vi "fsm_pluto_sequence_test.vi"() -> ()   [LabVIEW 2026]
uses:
  types/TestConfig.ctl
  <vilib>/Analysis/4window.llb/Hanning Window (DBL).vi
  <vilib>/Analysis/baseanly.llb/Mean (DBL).vi
  <vilib>/Analysis/2dsp.llb/Complex FFT.vi
  <vilib>/Analysis/4window.llb/AllCosWindow (DBL).vi
  <vilib>/Python/Open Venv Python Session.vi
  <vilib>/Analysis/1siggen.llb/Ramp Pattern by Samples.vi
  <vilib>/Analysis/NI_AALBase.lvlib
  <vilib>/Analysis/NI_AALPro.lvlib
panel:
  out "Received Signal \n Hann Windowed Spectrum":cluster{"Ramp Pattern":dbl[], dbl[]}(graph)
  out "Hann FFT Magnitude \nSpectrum (Normalized)":dbl[](array[numeric])
  out "Hann FFT Magnitude \nSpectrum (Centered)":dbl[](array[numeric])
  out "Hann FFT Magnitude\nSpectrum (Raw)":dbl[](array[numeric])
  out "Hann FFT \nComplex Spectrum":cdb[](array[numeric])
  out "Hann Windowed \nComplex Samples":cdb[](array[numeric])
  out "Windowed Q Samples":dbl[](array[numeric])
  out "Windowed I Samples":dbl[](array[numeric])
  out "FFT Magnitude Spectrum (Normalized)":dbl[](array[numeric])
  out "Received Signal \n Frequency Spectrum":cluster{"Ramp Pattern":dbl[], dbl[]}(graph)
  out "Frequency Axis (Mhz)":dbl[](array[numeric])
  out "FFT Magnitude Spectrum (Centered).":dbl[](array[numeric])
  out "N":i32
  out "FFT Magnitude Spectrum (Raw).":dbl[](array[numeric])
  out "FFT Complex Spectrum":cdb[](array[numeric])
  out "Raw Complex Samples":cdb[](array[numeric])
  out "Crest Factor (dB) indicator":dbl
  out "Crest Factor Valid":bool
  out "Crest Factor":dbl
  out "Peak Complex Magnitude":dbl
  out "Q RMS.":dbl
  out "I RMS.":dbl
  out "Q mean - DC offset":dbl format="%0.2f"
  out "I mean - DC offset":dbl format="%0.2f"
  out "Raw Q Samples":dbl[](array[numeric])
  out "Raw I Samples":dbl[](array[numeric])
  out "Sequence Index":i32
  out "Test Finished":bool
  out "Sequence Available":bool
  out "size(s)":i32
  out "Selected Configuration":T1
  in  "Test Sequence":T2(array[cluster])
  out "error out":errorcluster
  out "Acquisition Valid":bool
  out "Processing Valid":bool
  out "RMS Is Finite?":bool
  in  "Requested Samples":u32
  out "Capture Status":string
  out "Capture Configuration":string
  out "Error Status":string
  out "Resolved Log Path":path
  in  "Log File":path
  out "Log Record":string
  out "Log Status":string
  out "Processed Result":dbl
  out "Captured Data":dbl[](array[numeric])
  in  "Start Test":bool
  out "Current State":T3(ring)
  out "Configuration Status":string
  in  "Gain (dB)":dbl
  in  "Sample Rate (Ms/s)":dbl
  in  "Test Freq (Mhz)":dbl
  in  "stop":bool
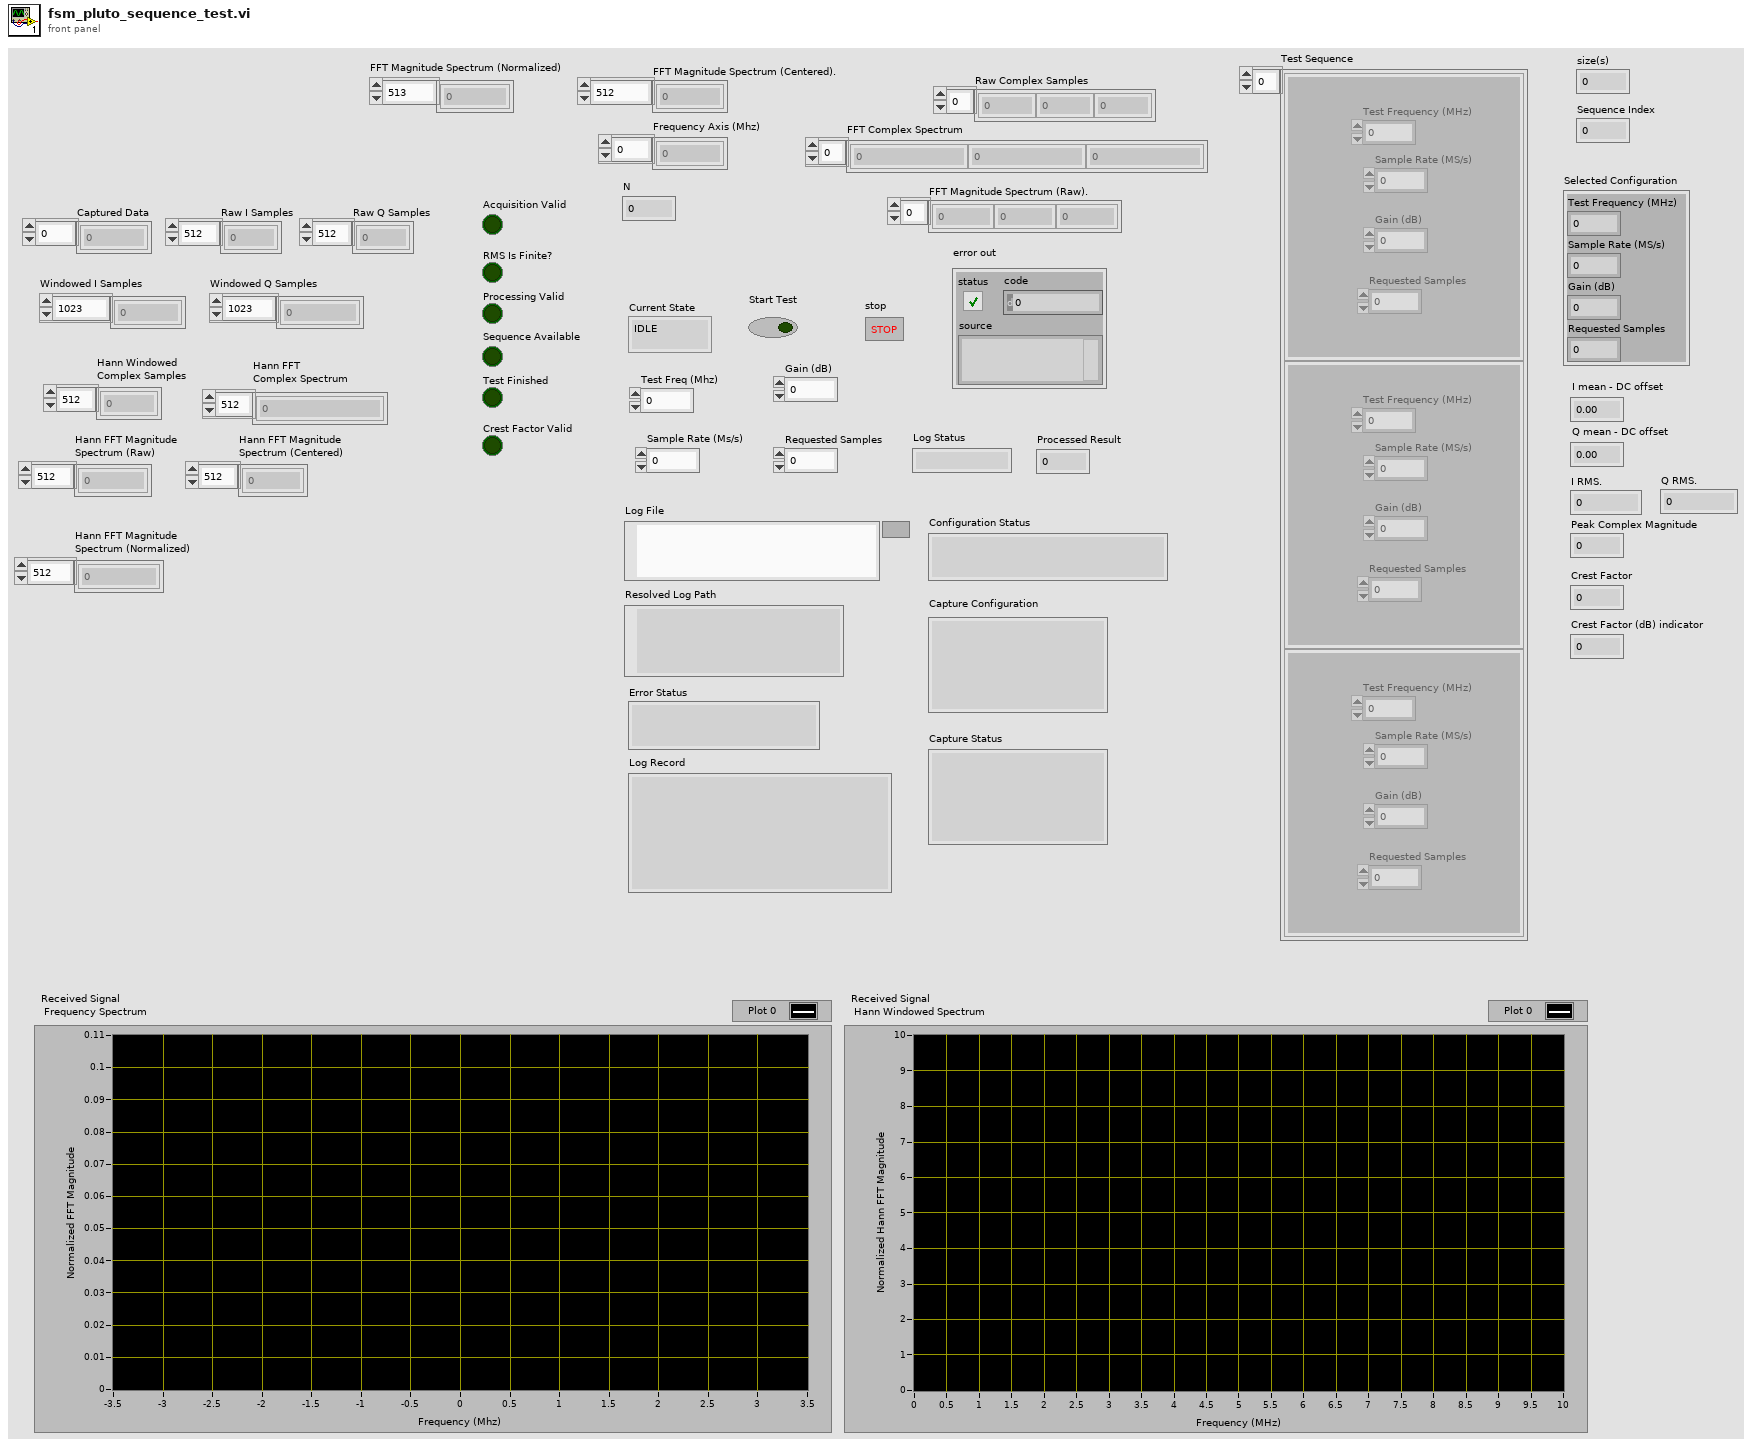
[diagram p1: front panel]
types:
  T1 = cluster{"Test Frequency (MHz)":dbl, "Sample Rate (MS/s)":dbl, "Gain (dB)":dbl, "Requested Samples":u32}
  T2 = cluster{"Test Frequency (MHz)":dbl, "Sample Rate (MS/s)":dbl, "Gain (dB)":dbl, "Requested Samples":u32}[]
  T3 = enum16{"IDLE", "CONFIGURE", "CAPTURE", "PROCESS", "LOG ", "ERROR "}
  T4 = cluster{"Acquisition Status":string, "Processing Status":string, "Overall Status":string, "Received Samples":u32, "RMS Value":dbl, "RMS Valid":bool, "Error Details":string}
  T5 = typedef "TestConfig.ctl" = cluster{"Test Frequency (Mhz)":dbl, "Sample Rate (Ms/s)":dbl, "Gain (dB)":dbl, "Requested Samples":u32}
  T6 = enum16{"open", "replace", "create", "open or create", "replace or create", "replace or create with confirmation"}
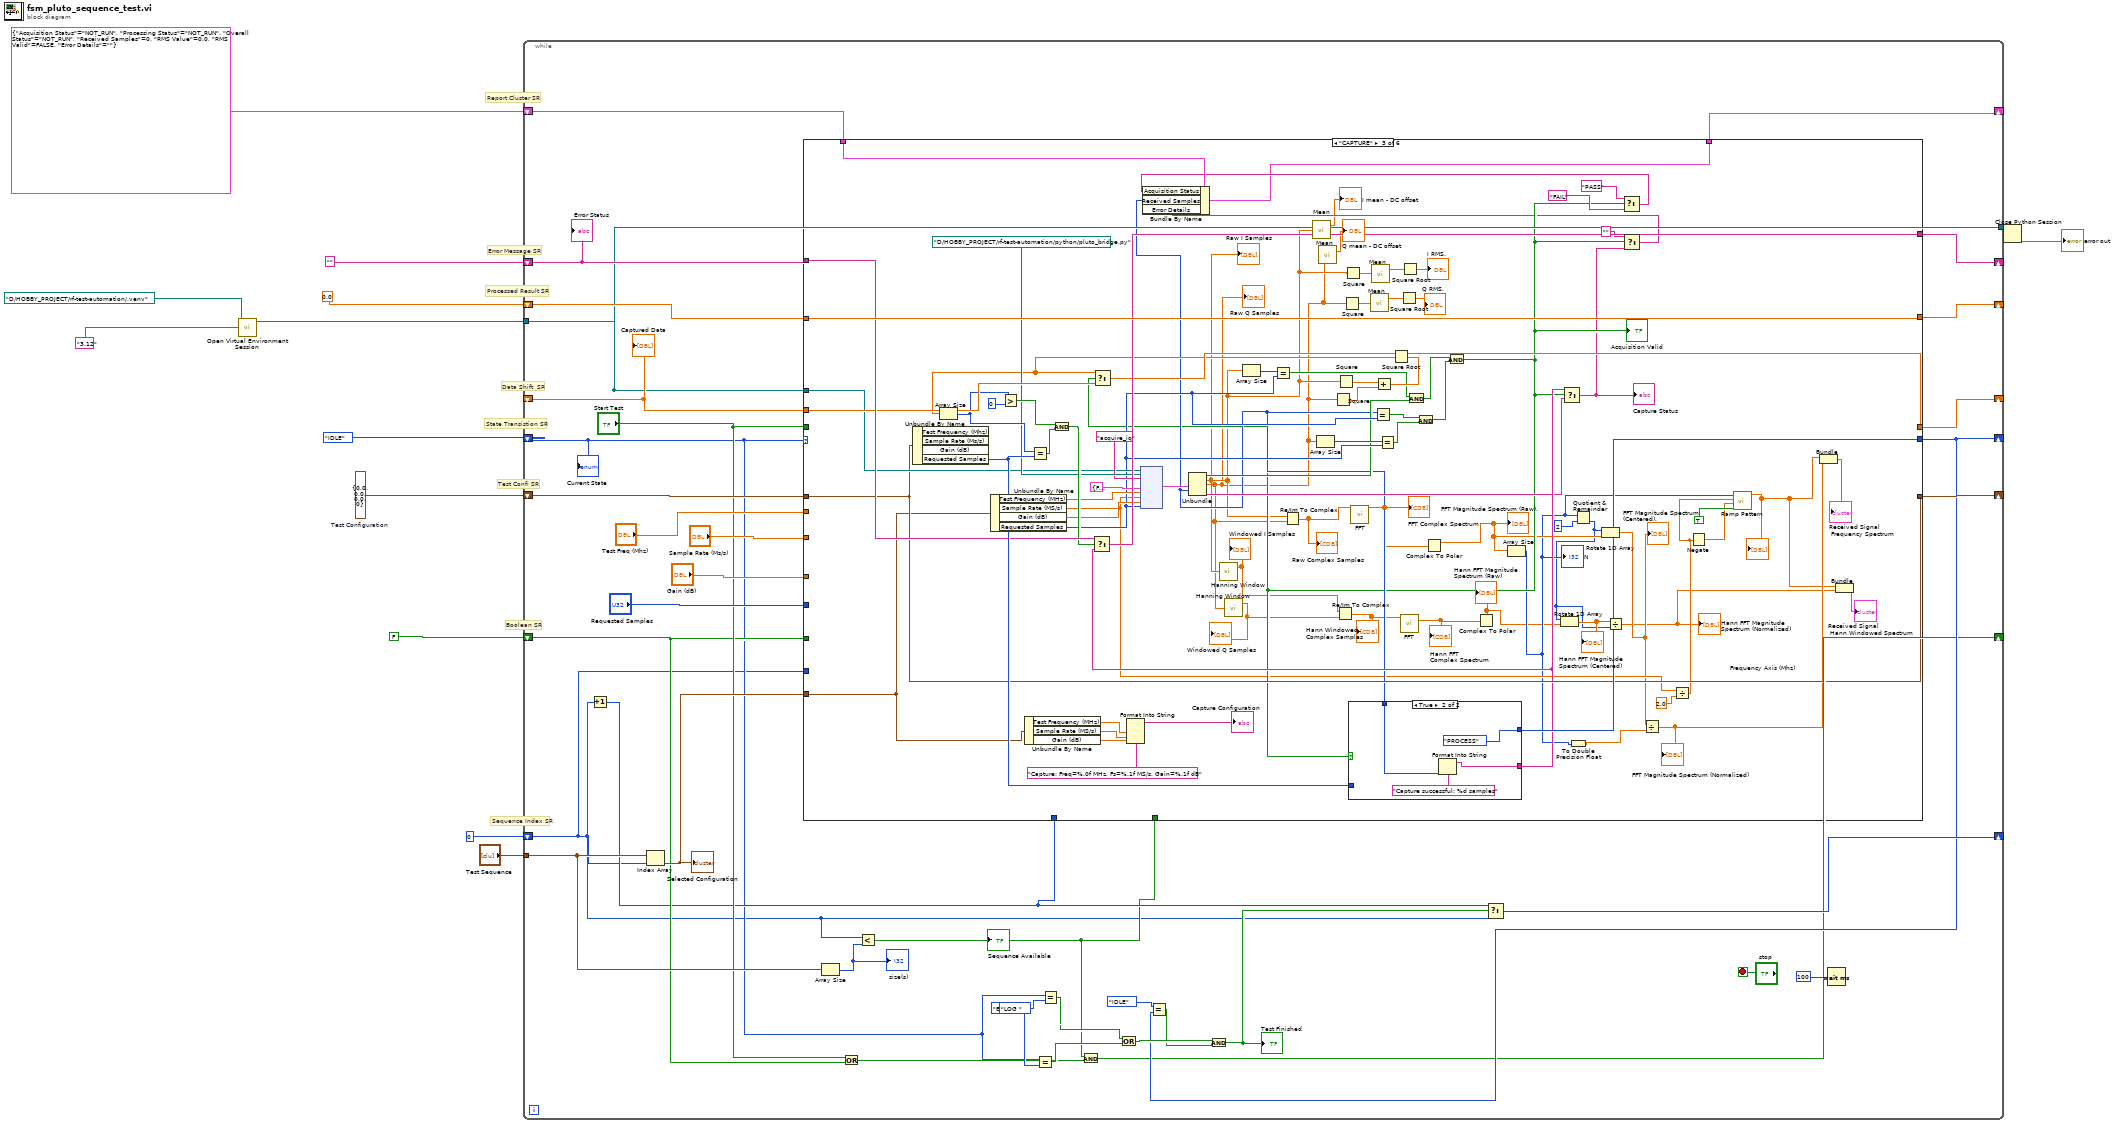
[diagram p0: block diagram]
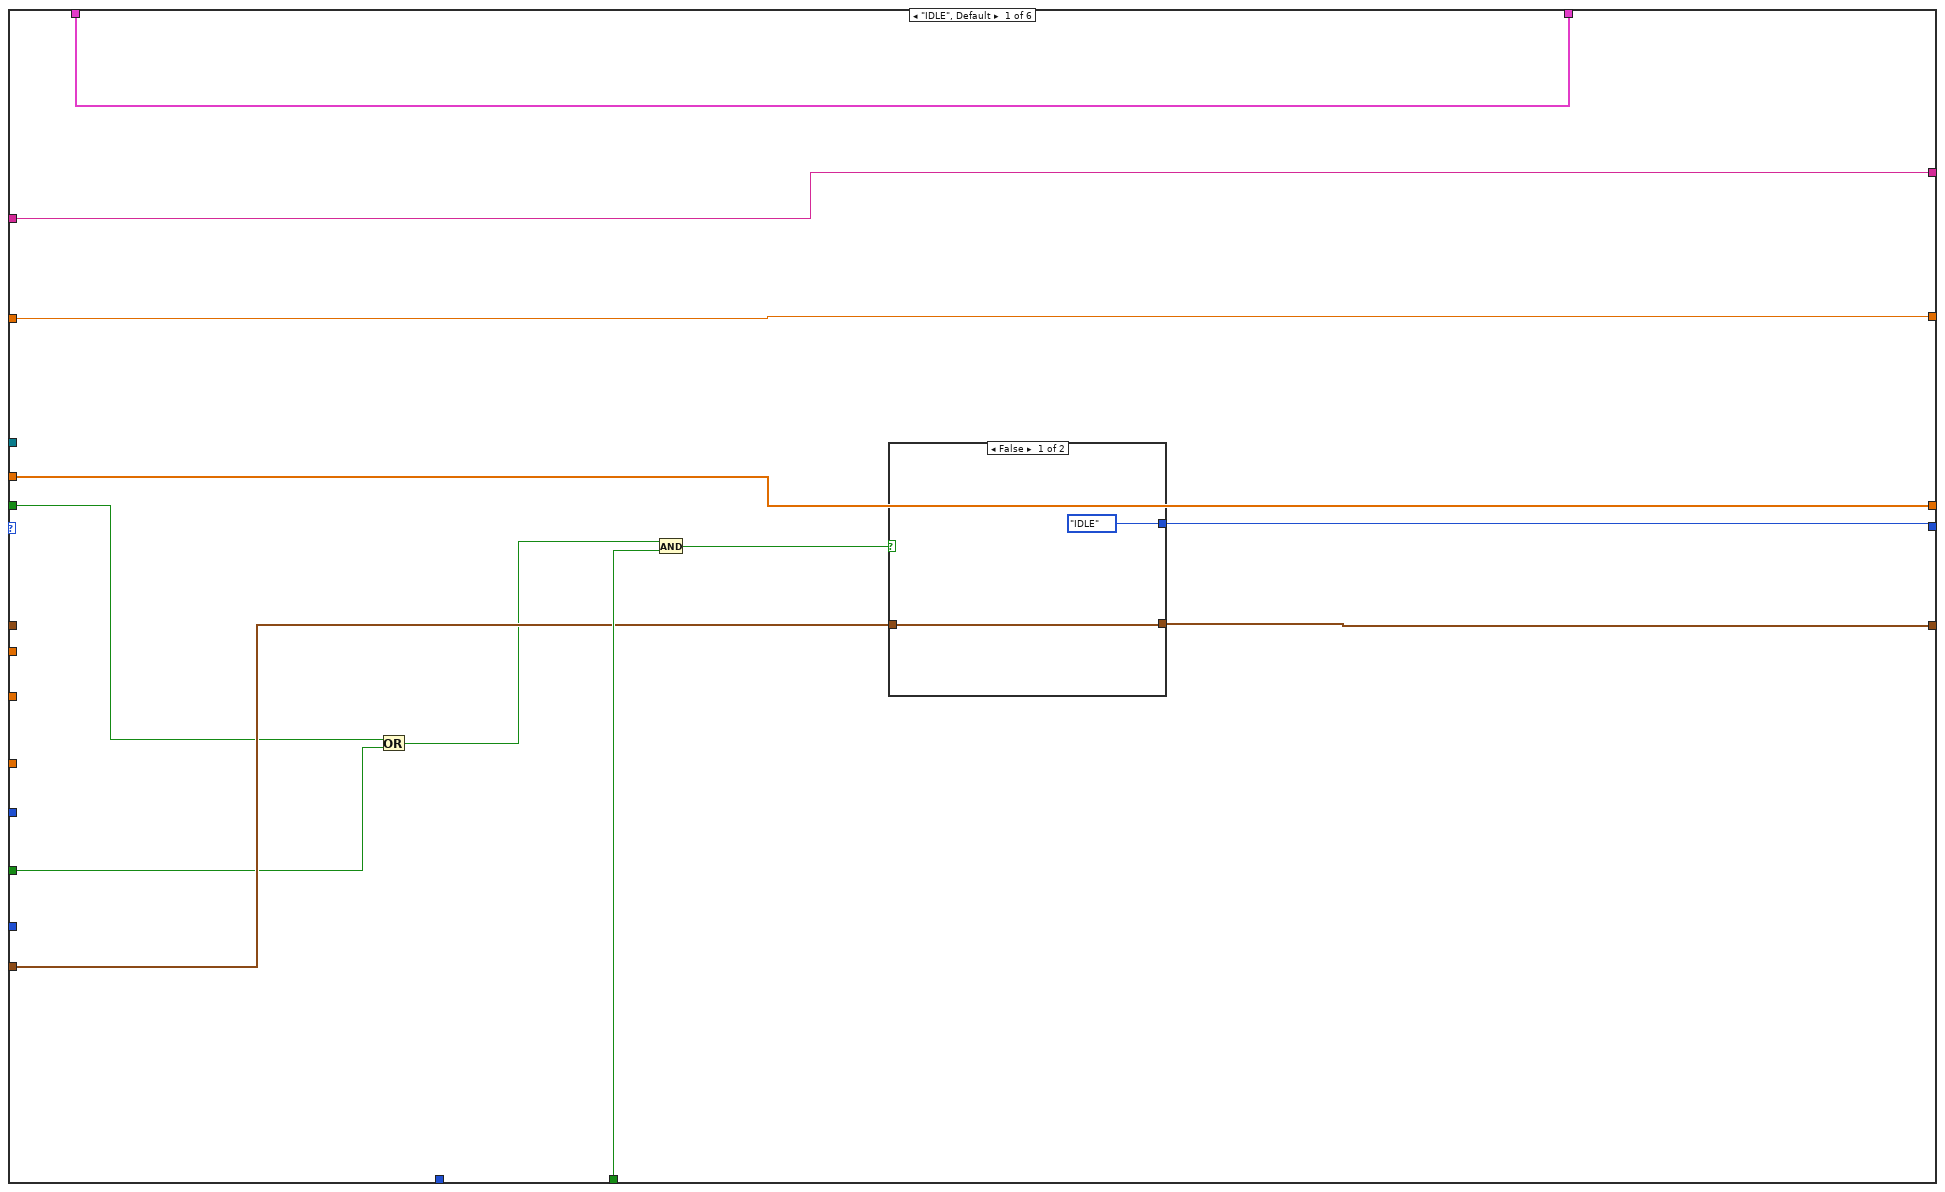
[diagram p2: hidden frame]
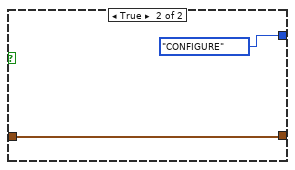
[diagram p3: hidden frame]
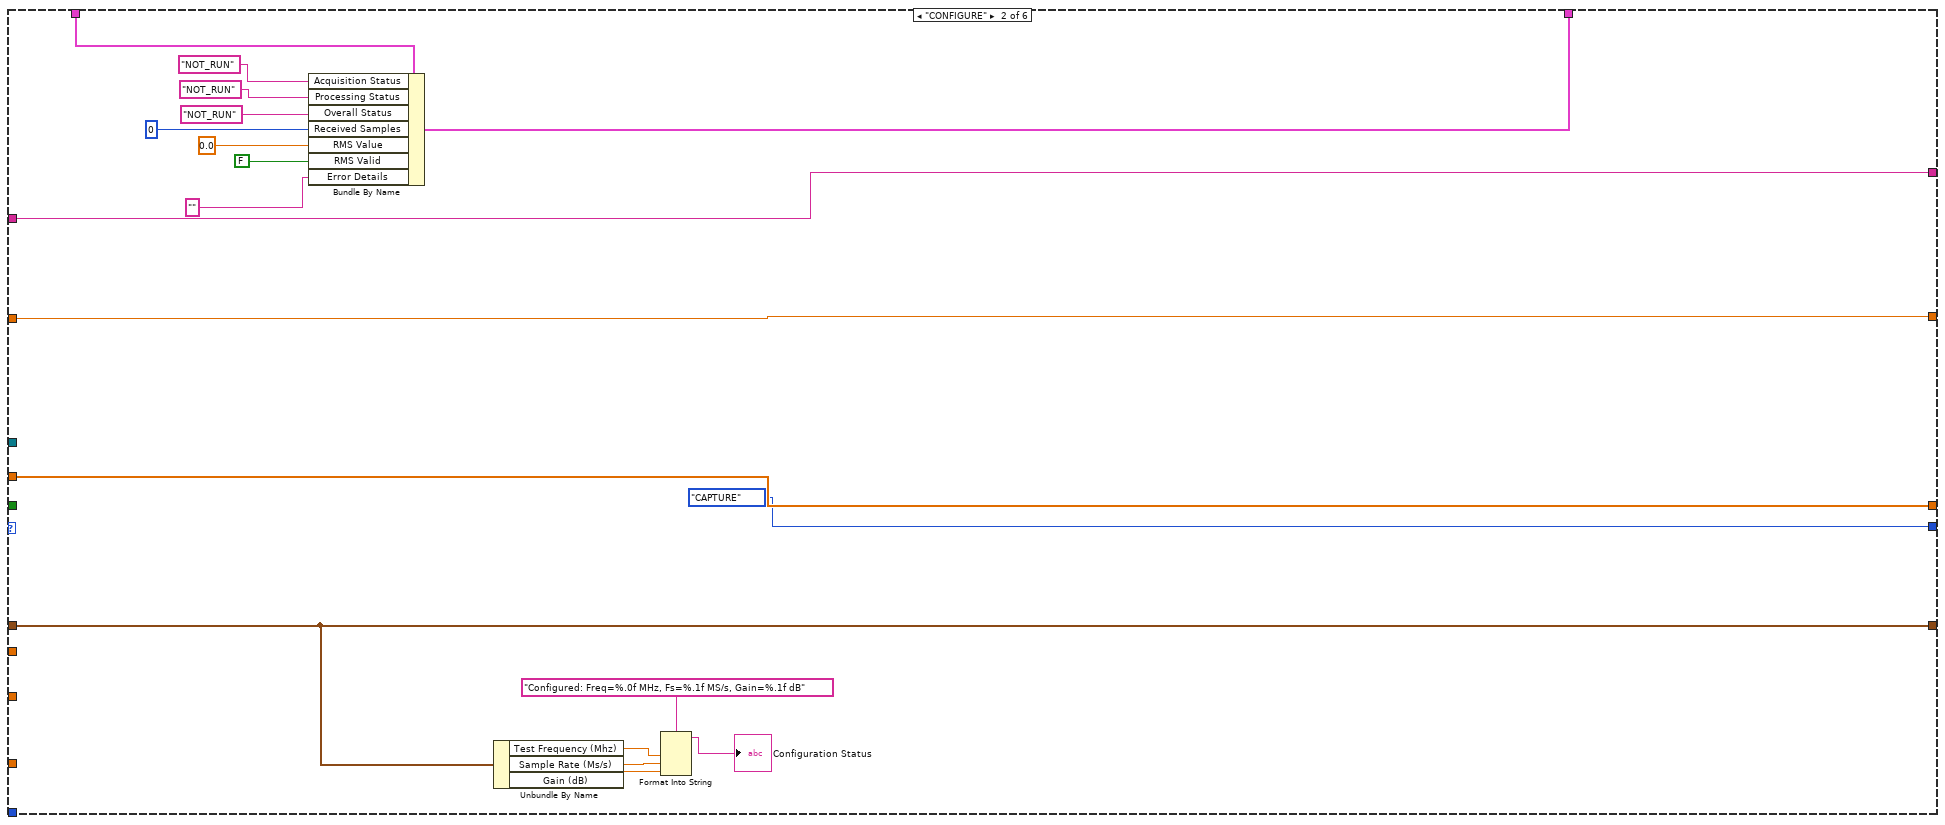
[diagram p4: hidden frame]
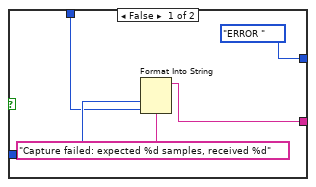
[diagram p5: hidden frame]
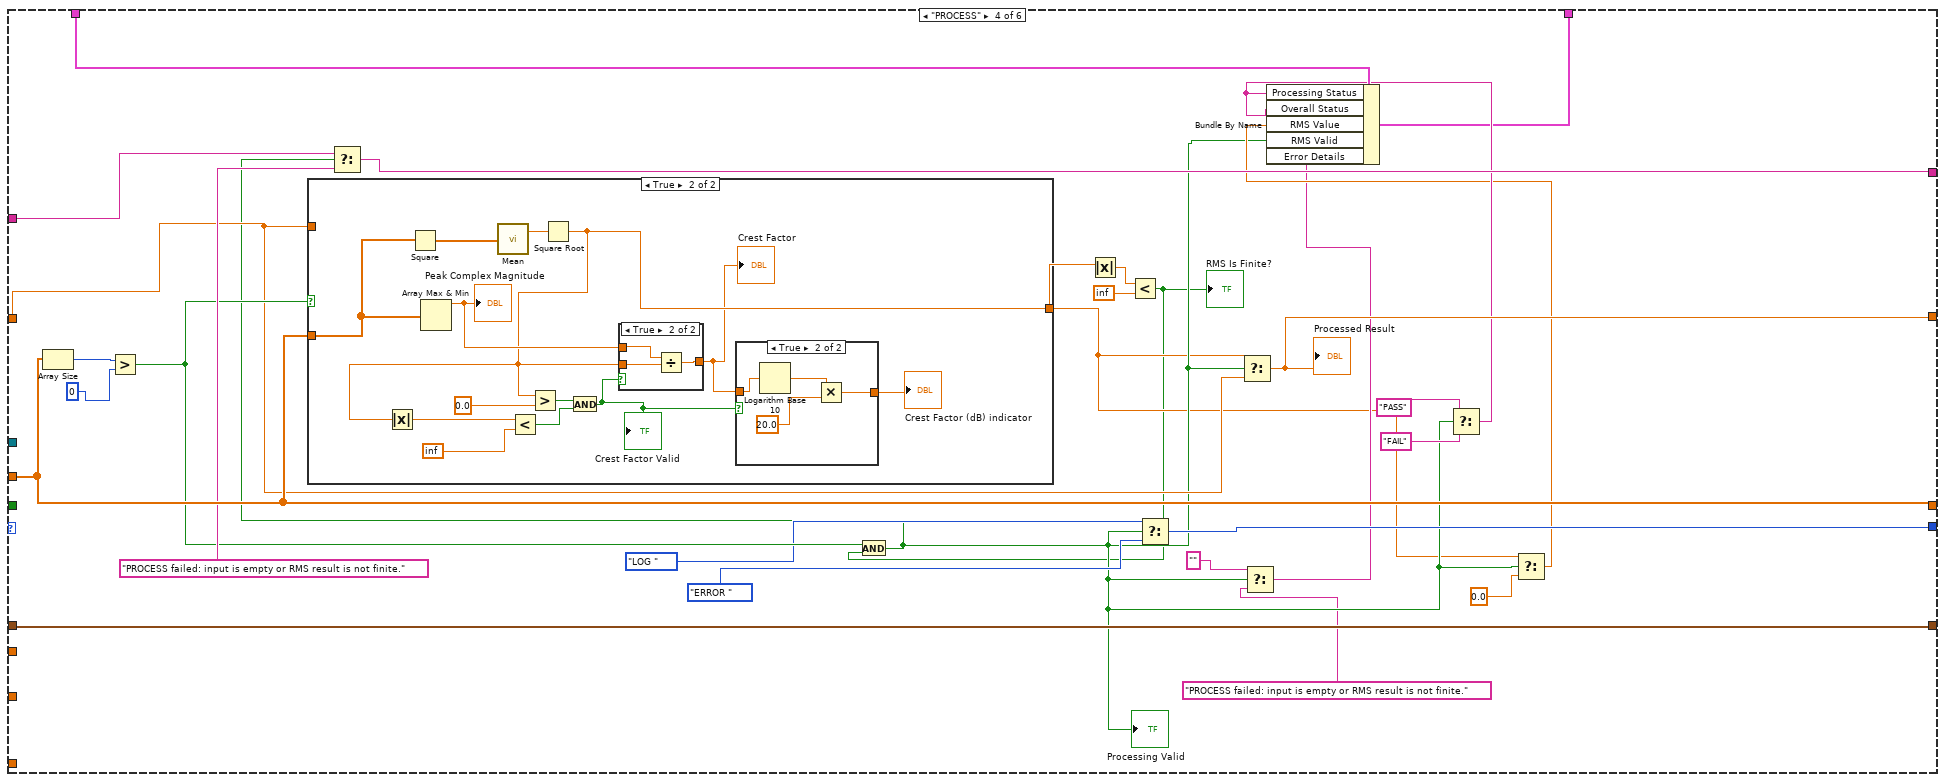
[diagram p6: hidden frame]
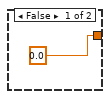
[diagram p8: hidden frame]
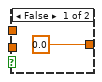
[diagram p9: hidden frame]
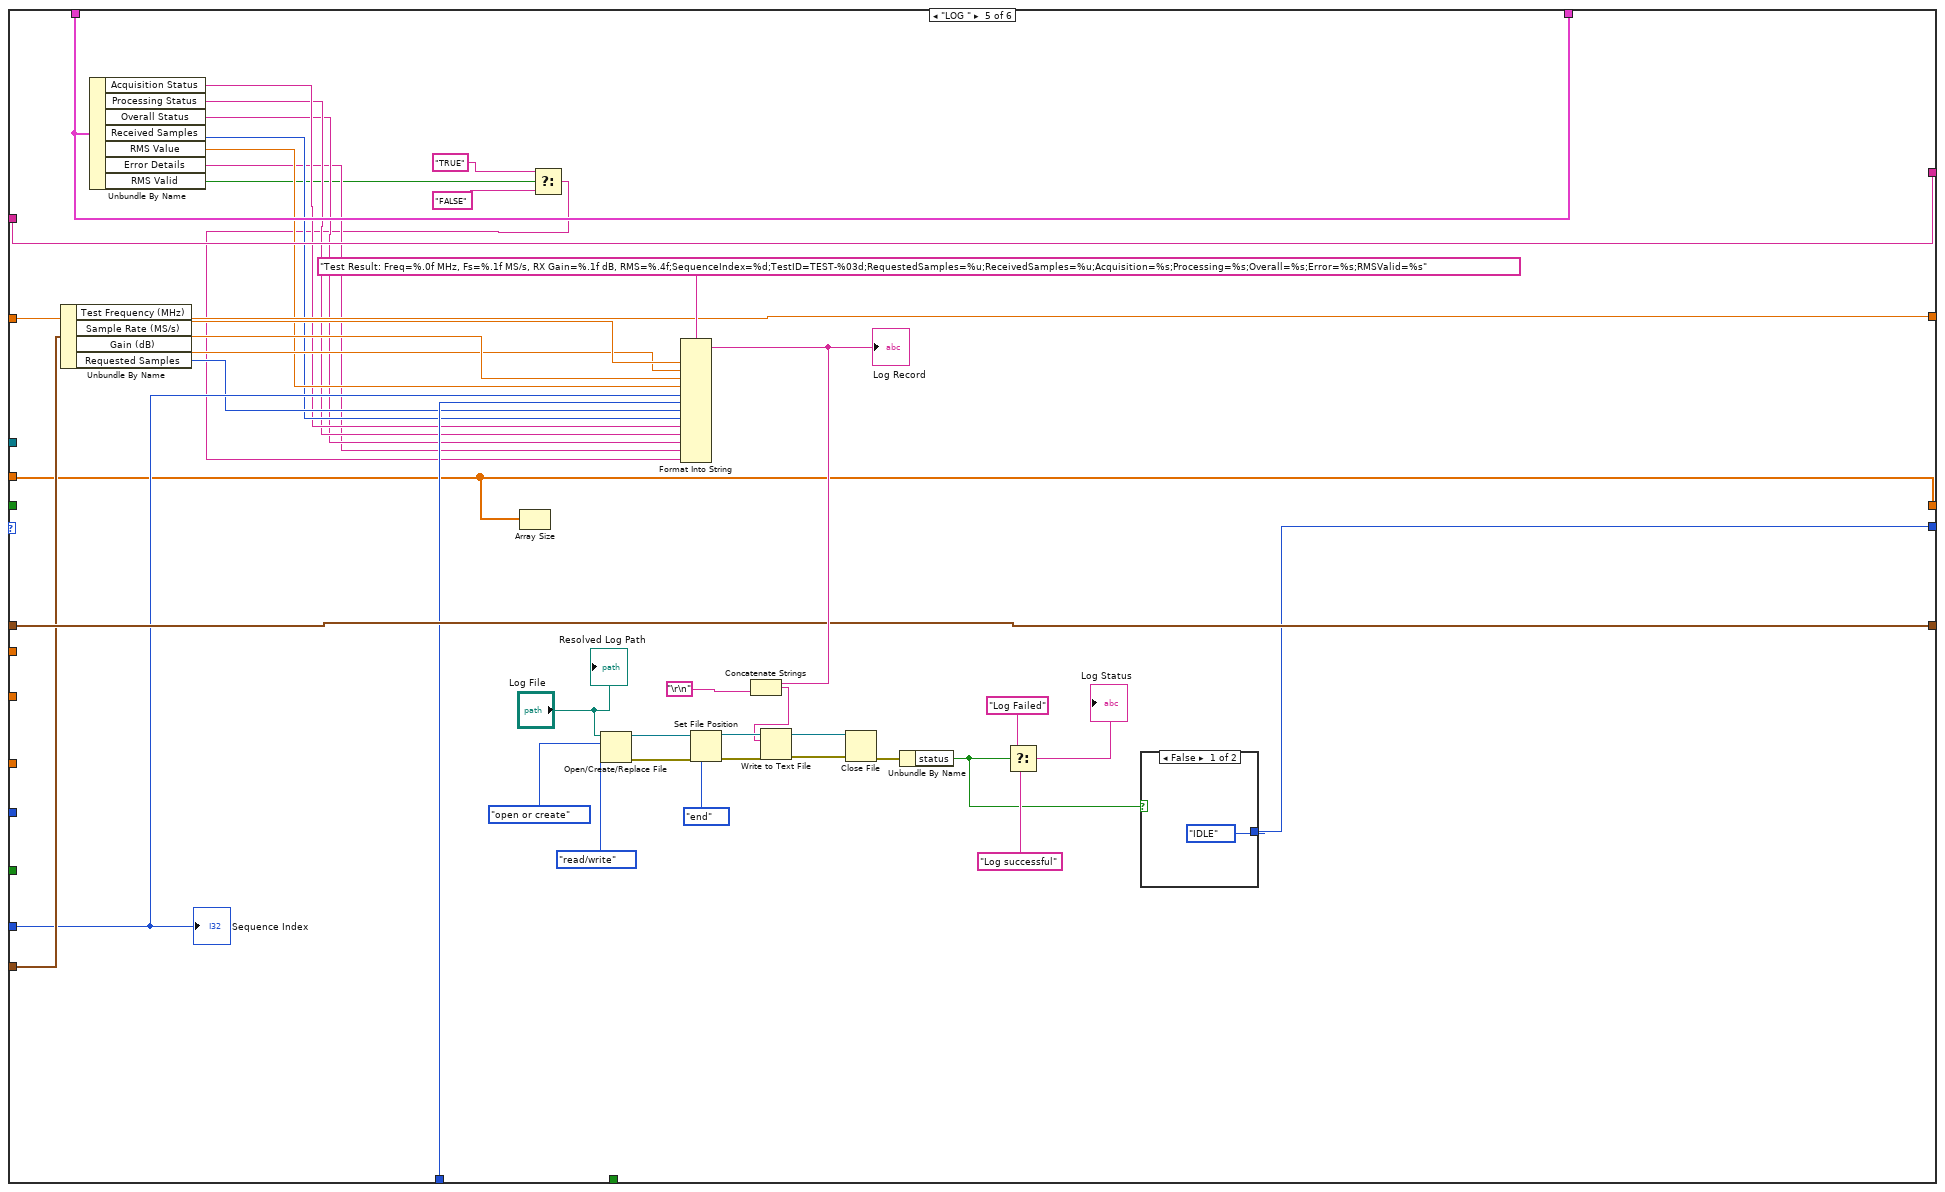
[diagram p10: hidden frame]
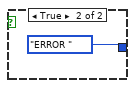
[diagram p11: hidden frame]
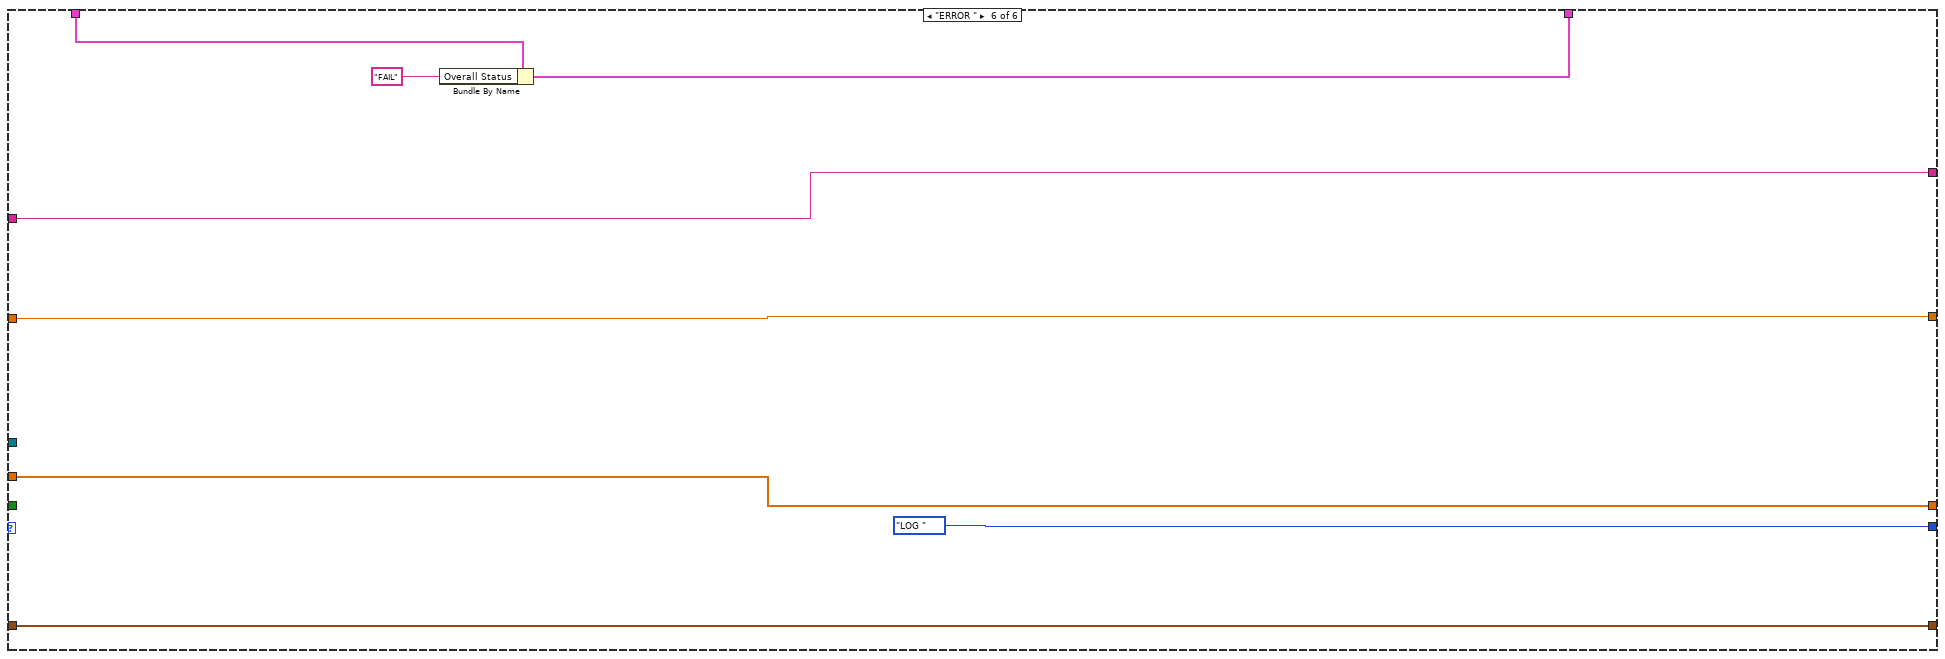
[diagram p12: hidden frame]
diagram:
  w10 = T5 {"Test Frequency (Mhz)"=0.0, "Sample Rate (Ms/s)"=0.0, "Gain (dB)"=0.0, "Requested Samples"=0}  # Test Configuration
  # "Sequence Index SR"
  # "Boolean SR"
  # "Test Confi SR"
  # "State Transistion SR"
  # "Data Shift  SR"
  # "Processed Result SR"
  # "Error Message SR"
  # "Report Cluster SR"
  n1 = call-poly <vilib>:"Open Virtual Environment Session.vi"("Python version"="3.12", "Env path"=path "D:/HOBBY_PROJECT/rf-test-automation/.venv") -> ("session out"=w7:refnum<k35>)  [unwired: 8 in, 1 out]
  n2 = while {
    shift-right: [w25] -> _
    shift-left: T3."IDLE" -> [w16]
    shift-right: [w49] -> _
    shift-left: _ -> [w48]
    shift-right: [w47] -> _
    shift-left: 0.0 -> [w46]
    shift-right: [w42] -> _
    shift-left: "" -> [w41]
    shift-right: [w39] -> _
    shift-left: w10 -> [w40]
    tunnel: w7 -> [w37]
    tunnel: [w37] -> w6
    shift-right: [w35] -> _
    shift-left: u32 0 -> [w14]
    tunnel: "Test Sequence" -> [w34]
    shift-right: [w21] -> _
    shift-left: FALSE -> [w23]
    shift-right: [w19] -> _
    shift-left: T4 {"Acquisition Status"="NOT_RUN", "Processing Status"="NOT_RUN", "Overall Status"="NOT_RUN", "Received Samples"=0, "RMS Value"=0.0, "RMS Valid"=FALSE, "Error Details"=""} -> [w18]
    stop <- "stop" stop-if-true
    n3 = Increment(x=w14) -> (x+1=w20:u32)
    n4 = Index Array(array=w34, index=w14) -> (element=w36:T1)
    "Selected Configuration" <- w36
    n5 = Array Size(array=w34) -> (size(s)=w33:i32)
    "size(s)" <- w33
    n6 = Or(x="Start Test", y=w23) -> (x .or. y?=w22:bool)
    n7 = Less?(x=w14, y=w33) -> (x < y?=w15:bool)
    "Sequence Available" <- w15
    n8 = case shown="\"CAPTURE\"" w16 {
      tunnel: "Test Freq (Mhz)" -> [_ _ _ _ _ _]
      tunnel: "Sample Rate (Ms/s)" -> [_ _ _ _ _ _]
      tunnel: "Gain (dB)" -> [_ _ _ _ _ _]
      tunnel: "Start Test" -> [w54 _ _ _ _ _]
      tunnel: [w63 w84 w160 w207 w243 w283] -> w49
      tunnel: w48 -> [w63 w84 w161 w207 w243 w283]
      tunnel: [w62 w83 w171 w196 w272 w282] -> w47
      tunnel: w46 -> [w62 w83 w171 w195 w272 w282]
      tunnel: [w61 T3."CAPTURE" w165 w197 w247 T3."LOG "] -> w25
      tunnel: [w60 w81 w162 w202 w253 w279] -> w42
      tunnel: w41 -> [w60 w81 w163 w204 w253 w279]
      tunnel: w40 -> [_ w80 w150 w208 w252 w280]
      tunnel: [w59 w80 w150 w208 w252 w280] -> w39
      tunnel: "Requested Samples" -> [_ _ _ _ _ _]
      tunnel: w37 -> [_ _ w151 _ _ _]
      tunnel: w36 -> [w56 _ w131 _ w251 _]
      tunnel: w15 -> [w57 _ _ _ _ _]
      tunnel: w23 -> [w55 _ _ _ _ _]
      tunnel: w14 -> [_ _ _ _ w246 _]
      tunnel: w20 -> [_ _ _ _ w245 _]
      tunnel: w18 -> [w52 w76 w130 w193 w242 w278]
      tunnel: [w52 w75 w121 w183 w242 w277] -> w19
      frame "IDLE", Default {
        n9 = Or(x=w54, y=w55) -> (x .or. y?=w53:bool)
        n10 = And(x=w53, y=w57) -> (x .and. y?=w58:bool)
        n11 = case shown="False" w58 {
          tunnel: [T3."IDLE" T3."CONFIGURE"] -> w61
          tunnel: [w64 w66] -> w59
          tunnel: w56 -> [w64 w66]
          frame False {
          }
          frame True {
          }
        }
      }
      frame "CONFIGURE" {
        n12 = Bundle By Name(cluster=w76, "Acquisition Status"="NOT_RUN", "Processing Status"="NOT_RUN", "Overall Status"="NOT_RUN", "Received Samples"=0, "RMS Value"=0.0, "RMS Valid"=FALSE, "Error Details"="") -> (w75:T4)
        n13 = Unbundle By Name(w80) -> ("Test Frequency (Mhz)"=w79:dbl, "Sample Rate (Ms/s)"=w78:dbl, "Gain (dB)"=w77:dbl)
        n14 = Format Into String(format string="Configured: Freq=%.0f MHz, Fs=%.1f MS/s, Gain=%.1f dB", w79, w78, w77) -> (resulting string=→"Configuration Status":string)  [unwired: 2 in, 1 out]
      }
      frame "CAPTURE" {
        n15 = Unbundle By Name(w150) -> ("Requested Samples"=w164:u32)  [unwired: 3 out]
        n16 = Unbundle By Name(w131) -> ("Test Frequency (MHz)"=w149:dbl, "Sample Rate (MS/s)"=w108:dbl, "Gain (dB)"=w148:dbl, "Requested Samples"=w141:u32)
        n17 = Unbundle By Name(w131) -> ("Test Frequency (MHz)"=w169:dbl, "Sample Rate (MS/s)"=w168:dbl, "Gain (dB)"=w167:dbl)
        n18 = Format Into String(format string="Capture: Freq=%.0f MHz, Fs=%.1f MS/s, Gain=%.1f dB", w169, w168, w167) -> (resulting string=→"Capture Configuration":string)  [unwired: 2 in, 1 out]
        n19 = node(w151, path "D:/HOBBY_PROJECT/rf-test-automation/python/pluto_bridge.py" ("module path"), "acquire_iq" ("function name"), cluster{bool, dbl[], dbl[], i32, string} {FALSE, [], [], 0, ""}, w149, w108, w148, w141) -> (w147:cluster{bool, dbl[], dbl[], i32, string})  [unwired: 5 in, 4 out]
        n20 = Unbundle(w147) -> (w139:bool, w98:dbl[], w97:dbl[], w126:i32, w132:string)
        "Raw I Samples" <- w98
        "Raw Q Samples" <- w97
        n21 = call-poly <vilib>:"Hanning Window.vi"("X"=w98) -> ("Windowed X"=w96:dbl[])  [unwired: 1 out]
        "Windowed I Samples" <- w96
        n22 = call-poly <vilib>:"Hanning Window.vi"("X"=w97) -> ("Windowed X"=w95:dbl[])  [unwired: 1 out]
        "Windowed Q Samples" <- w95
        n23 = Array Size(array=w98) -> (size(s)=w142:i32)
        n24 = Equal?(x=w142, y=w141) -> (x = y?=w140:bool)
        n25 = Re/Im To Complex(1:w97, 2:w98) -> (0:w112:cdb[])
        "Raw Complex Samples" <- w112
        n26 = call-poly <vilib>:"Mean.vi"("X"=w98) -> ("mean"=→"I mean - DC offset":dbl)  [unwired: 1 out]
        n27 = Array Size(array=w97) -> (size(s)=w143:i32)
        n28 = call-poly <vilib>:"Mean.vi"("X"=w97) -> ("mean"=→"Q mean - DC offset":dbl)  [unwired: 1 out]
        n29 = Square(x=w97) -> (x^2=w146:dbl[])
        n30 = Re/Im To Complex(1:w95, 2:w96) -> (0:w94:cdb[])
        "Hann Windowed \nComplex Samples" <- w94
        n31 = Square(x=w98) -> (x^2=w145:dbl[])
        n32 = Square(x=w97) -> (x^2=w117:dbl[])
        n33 = Square(x=w98) -> (x^2=w116:dbl[])
        n34 = call-poly <vilib>:"FFT.vi"("X"=w112) -> ("FFT {X}"=w111:cdb[])  [unwired: 9 in, 1 out]
        "FFT Complex Spectrum" <- w111
        n35 = call-poly <vilib>:"Mean.vi"("X"=w117) -> ("mean"=w115:dbl)  [unwired: 1 out]
        n36 = call-poly <vilib>:"Mean.vi"("X"=w116) -> ("mean"=w118:dbl)  [unwired: 1 out]
        n37 = Equal?(x=w126, y=w141) -> (x = y?=w138:bool)
        n38 = Add(x=w145, y=w146) -> (x+y=w144:dbl[])
        n39 = Equal?(x=w143, y=w141) -> (x = y?=w137:bool)
        n40 = Square Root(x=w144) -> (sqrt(x)=w134:dbl[])
        n41 = Array Size(array=w134) -> (size(s)=w156:i32)
        n42 = Greater?(x=w156, y=0) -> (0:w159:bool)
        n43 = Equal?(x=w156, y=w164) -> (x = y?=w158:bool)
        n44 = And(x=w159, y=w158) -> (x .and. y?=w157:bool)
        n45 = Square Root(x=w115) -> (sqrt(x)=→"Q RMS.":dbl)
        n46 = call-poly <vilib>:"FFT.vi"("X"=w94) -> ("FFT {X}"=w93:cdb[])  [unwired: 9 in, 1 out]
        "Hann FFT \nComplex Spectrum" <- w93
        n47 = Square Root(x=w118) -> (sqrt(x)=→"I RMS.":dbl)
        n48 = And(x=w140, y=w139) -> (x .and. y?=w136:bool)
        n49 = And(x=w138, y=w137) -> (x .and. y?=w135:bool)
        n50 = Complex To Polar(r * e^(i*theta)=w111) -> (r=w110:dbl[])  [unwired: 1 out]
        "FFT Magnitude Spectrum (Raw)." <- w110
        n51 = And(x=w136, y=w135) -> (x .and. y?=w125:bool)
        "Acquisition Valid" <- w125
        n52 = Select(t=w134, s=w125, f=w161) -> (s? t:f=w160:dbl[])
        n53 = case shown="True" w125 {
          tunnel: [T3."ERROR " T3."PROCESS"] -> w165
          tunnel: w164 -> [w174 _]
          tunnel: [w173 w179] -> w133
          tunnel: w126 -> [w172 w177]
          frame False {
            n54 = Format Into String(format string="Capture failed: expected %d samples, received %d", w174, w172) -> (resulting string=w173:string)  [unwired: 2 in, 1 out]
          }
          frame True {
            n55 = Format Into String(format string="Capture successful: %d samples", w177) -> (resulting string=w179:string)  [unwired: 2 in, 1 out]
          }
        }
        n56 = Select(t=w163, s=w157, f=w133) -> (s? t:f=w162:string)
        n57 = Complex To Polar(r * e^(i*theta)=w93) -> (r=w92:dbl[])  [unwired: 1 out]
        "Hann FFT Magnitude\nSpectrum (Raw)" <- w92
        n58 = Array Size(array=w110) -> (size(s)=w101:i32)
        "N" <- w101
        n59 = Select(t=w133, s=w125, f=w132) -> (s? t:f=w123:string)
        "Capture Status" <- w123
        n60 = To Double Precision Float(number=w101) -> (double precision float=w100:dbl)
        n61 = Quotient & Remainder(x=w101, y=2) -> (floor(x/y)=w90:i32)  [unwired: 1 out]
        n62 = Rotate 1D Array(1:w92, 2:w90) -> (0:w91:dbl[])
        "Hann FFT Magnitude \nSpectrum (Centered)" <- w91
        n63 = Rotate 1D Array(1:w110, 2:w90) -> (0:w103:dbl[])
        "FFT Magnitude Spectrum (Centered)." <- w103
        n64 = Divide(x=w91, y=w90) -> (x/y=w88:dbl[])
        "Hann FFT Magnitude \nSpectrum (Normalized)" <- w88
        n65 = Select(t="PASS", s=w125, f="FAIL") -> (s? t:f=w127:string)
        n66 = Select(t="", s=w125, f=w123) -> (s? t:f=w122:string)
        n67 = Bundle By Name(cluster=w130, "Acquisition Status"=w127, "Received Samples"=w126, "Error Details"=w122) -> (w121:T4)
        n68 = Divide(x=w103, y=w100) -> (x/y=w99:dbl[])
        "FFT Magnitude Spectrum (Normalized)" <- w99
        n69 = Divide(x=w108, y=2.0) -> (x/y=w102:dbl)
        n70 = Negate(x=w102) -> (-x=w105:dbl)
        n71 = call-poly <vilib>:"Ramp Pattern.vi"("exclude end?"=TRUE, "start"=w105, "end"=w102, "samples"=w101) -> ("Ramp Pattern"=w89:dbl[])  [unwired: 6 in, 1 out]
        "Frequency Axis (Mhz)" <- w89
        n72 = Bundle("Ramp Pattern"=w89, w99) -> (→"Received Signal \n Frequency Spectrum":cluster{"Ramp Pattern":dbl[], dbl[]})  [unwired: 1 in]
        n73 = Bundle("Ramp Pattern"=w89, w88) -> (→"Received Signal \n Hann Windowed Spectrum":cluster{"Ramp Pattern":dbl[], dbl[]})  [unwired: 1 in]
      }
      frame "PROCESS" {
        n74 = Array Size(array=w207) -> (size(s)=w206:i32)
        n75 = Greater?(x=w206, y=0) -> (0:w200:bool)
        n76 = case shown="True" w200 {
          tunnel: [w209 w213] -> w182
          tunnel: w207 -> [_ w220]
          tunnel: w195 -> [w209 _]
          frame False {
          }
          frame True {
            n77 = Square(x=w220) -> (x^2=w222:dbl[])
            n78 = Array Max & Min(array=w220) -> (max value=w214:dbl)  [unwired: 3 out]
            "Peak Complex Magnitude" <- w214
            n79 = call-poly <vilib>:"Mean.vi"("X"=w222) -> ("mean"=w221:dbl)  [unwired: 1 out]
            n80 = Square Root(x=w221) -> (sqrt(x)=w213:dbl)
            n81 = Absolute Value(x=w213) -> (abs(x)=w217:dbl)
            n82 = Less?(x=w217, y=inf) -> (x < y?=w215:bool)
            n83 = Greater?(x=w213, y=0.0) -> (0:w218:bool)
            n84 = And(x=w218, y=w215) -> (x .and. y?=w212:bool)
            "Crest Factor Valid" <- w212
            n85 = case shown="True" w212 {
              tunnel: w214 -> [_ w231]
              tunnel: w213 -> [_ w230]
              tunnel: [0.0 w229] -> w211
              frame False {
              }
              frame True {
                n86 = Divide(x=w231, y=w230) -> (x/y=w229:dbl)
              }
            }
            "Crest Factor" <- w211
            n87 = case shown="True" w212 {
              tunnel: w211 -> [_ w227]
              tunnel: [0.0 w224] -> w210
              frame False {
              }
              frame True {
                n88 = Logarithm Base 10(1:w227) -> (0:w226:dbl)
                n89 = Multiply(x=w226, y=20.0) -> (x*y=w224:dbl)
              }
            }
            "Crest Factor (dB) indicator" <- w210
          }
        }
        n90 = Absolute Value(x=w182) -> (abs(x)=w201:dbl)
        n91 = Less?(x=w201, y=inf) -> (x < y?=w181:bool)
        "RMS Is Finite?" <- w181
        n92 = And(x=w200, y=w181) -> (x .and. y?=w187:bool)
        "Processing Valid" <- w187
        n93 = Select(t=w204, s=w187, f="PROCESS failed: input is empty or RMS result is not finite.") -> (s? t:f=w202:string)
        n94 = Select(t=T3."LOG ", s=w187, f=T3."ERROR ") -> (s? t:f=w197:T3)
        n95 = Select(t=w182, s=w187, f=w195) -> (s? t:f=w196:dbl)
        "Processed Result" <- w196
        n96 = Select(t="" ("f"), s=w187, f="PROCESS failed: input is empty or RMS result is not finite.") -> (s? t:f=w184:string)
        n97 = Select(t="PASS" ("f"), s=w187, f="FAIL") -> (s? t:f=w190:string)
        n98 = Select(t=w182, s=w187, f=0.0) -> (s? t:f=w188:dbl)
        n99 = Bundle By Name(cluster=w193, "Processing Status"=w190, "Overall Status"=w190, "RMS Value"=w188, "RMS Valid"=w187, "Error Details"=w184) -> (w183:T4)
      }
      frame "LOG " {
        n100 = Unbundle By Name(w251) -> ("Test Frequency (MHz)"=w249:dbl, "Sample Rate (MS/s)"=w248:dbl, "Gain (dB)"=w250:dbl, "Requested Samples"=w244:u32)
        n101 = Unbundle By Name(w242) -> ("Acquisition Status"=w239:string, "Processing Status"=w238:string, "Overall Status"=w237:string, "Received Samples"=w240:u32, "RMS Value"=w241:dbl, "Error Details"=w236:string, "RMS Valid"=w235:bool)
        n102 = Array Size(array=w243) -> ()  [unwired: 1 out]
        n103 = Select(t="TRUE", s=w235, f="FALSE" ("t")) -> (s? t:f=w232:string)
        n104 = Open/Create/Replace File(file path (use dialog)="Log File", operation (0:open)=T6."open or create", access (0:read/write)=enum16{"read/write", "read-only", "write-only"}."read/write") -> (refnum out=w271:refnum<file>, error out=w266:errorcluster)  [unwired: 3 in, 1 out]
        n105 = Format Into String(format string="Test Result: Freq=%.0f MHz, Fs=%.1f MS/s, RX Gain=%.1f dB, RMS=%.4f;SequenceIndex=%d;TestID=TEST-%03d;RequestedSamples=%u;ReceivedSamples=%u;Acquisition=%s;Processing=%s;Overall=%s;Error=%s;RMSValid=%s", w249, w248, w250, w241, w246, w245, w244, w240, w239, w238, w237, w236, w232) -> (resulting string=w269:string)  [unwired: 2 in, 1 out]
        "Log Record" <- w269
        n106 = Set File Position(refnum=w271, from (0:start)=enum16{"start", "end", "current"}."end", error in=w266) -> (refnum out=w270:refnum<file>, error out=w265:errorcluster)  [unwired: 1 in]
        n107 = Concatenate Strings(w269, "\r\n") -> (w256:string)
        n108 = Write to Text File(file (use dialog)=w270, text=w256, error in=w265) -> (refnum out=w267:refnum<file>, error out=w264:errorcluster)  [unwired: 1 in, 1 out]
        n109 = Close File(refnum=w267, error in=w264) -> (error out=w263:errorcluster)  [unwired: 1 out]
        n110 = Unbundle By Name(w263) -> ("status"=w254:bool)
        n111 = Select(t="Log Failed", s=w254, f="Log successful") -> (s? t:f=→"Log Status":string)
        n112 = case shown="False" w254 {
          tunnel: [T3."IDLE" T3."ERROR "] -> w247
          frame False {
          }
          frame True {
          }
        }
        "Resolved Log Path" <- "Log File"
        "Sequence Index" <- w246
      }
      frame "ERROR " {
        n113 = Bundle By Name(cluster=w278, "Overall Status"="FAIL") -> (w277:T4)
      }
    }
    n114 = Equal?(x=w16, y=T3."ERROR ") -> (x = y?=w31:bool)
    n115 = Equal?(x=w16, y=T3."LOG ") -> (x = y?=w32:bool)
    n116 = And(x=w15, y=w22) -> (x .and. y?=w21:bool)
    n117 = Or(x=w32, y=w31) -> (x .or. y?=w27:bool)
    n118 = Equal?(x=T3."IDLE", y=w25) -> (x = y?=w26:bool)
    n119 = And(x=w27, y=w26) -> (x .and. y?=w17:bool)
    "Test Finished" <- w17
    n120 = Select(t=w20, s=w17, f=w14) -> (s? t:f=w35:u32)
    n121 = Wait (ms)(milliseconds to wait=u32 100) -> ()  [unwired: 1 out]
    "Current State" <- w16
    "Captured Data" <- w48
    "Error Status" <- w41
  }
  n122 = Close Python Session(session in=w6) -> (11:→"error out":errorcluster)  [unwired: 1 in]
